vi "New (Single Trigger).vi"(6 "file name format (\"logfile_%<%Y-%m-%d_%H-%M-%S>T.log\")":string="logfile_%<%Y-%m-%d_%H-%M-%S>T.log", 7 "cleanup filter (never)":refnum<class "CleanupFilter.lvclass">, 8 "error in":errorcluster, 9 "rollover trigger (50 MB)":refnum<class "RolloverTrigger.lvclass">, 10 "formatter (JSON)":refnum<class "Formatter.lvclass">, 11 "log directory (<app dir>/logs)":path) -> (0 "error out":errorcluster, 2 "events":T1, 3 "file handler":refnum<class "File Handler.lvclass">)   [LabVIEW 2018, in "GLog.lvlib" / "File Handler.lvclass"]
doc: "Creates a new Handler which writes log records to a file."
uses:
  File Handler.lvclass
  C:/Users/Colin/Documents/software_projects/labview/glog/src/api/extension/formatting_handler_interface/Formatting Handler.lvclass
  extension/formatter_interface/Formatter.lvclass
  RolloverTrigger/RolloverTrigger.lvclass
  Events.ctl
  File Update Event.ctl
  CleanupFilter/CleanupFilter.lvclass
  File Handler.lvclass/File Handler.ctl
  extension/formatting_handler_interface/Formatting Handler.lvclass/Formatting Handler.ctl
  RolloverTrigger.Size/RolloverTrigger.Size.lvclass
  C:/Users/Colin/Documents/software_projects/labview/glog/src/api/configuration/handlers/file_handler/RolloverTrigger/RolloverTrigger.lvclass
  formatters/JSON_formatter/JSON.lvclass
  C:/Users/Colin/Documents/software_projects/labview/glog/src/api/extension/formatter_interface/Formatter.lvclass
  extension/formatting_handler_interface/Formatting Handler.lvclass
panel:
  # "Connector Pane"
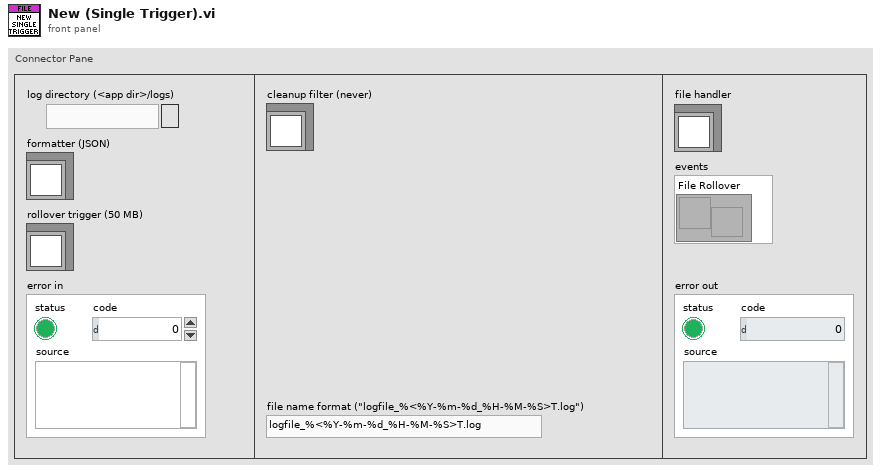
[diagram p1: front panel]
types:
  T1 = typedef "GLog.lvlib/File Handler.lvclass/Events.ctl" = cluster{"File Rollover":refnum<user-event>}
  T2 = typedef "GLog.lvlib/File Handler.lvclass/File Update Event.ctl" = cluster{"Current File":path, "Source":string}
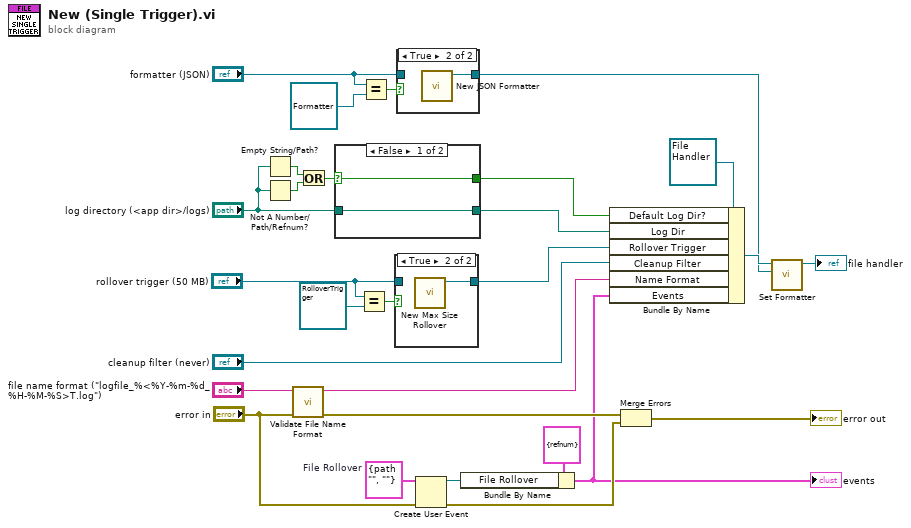
[diagram p0: block diagram]
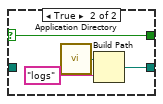
[diagram p4: hidden frame]
diagram:
  w16 = T2 {"Current File"=path "", "Source"=""}  # File Rollover
  n1 = Empty String/Path?(string/path="log directory (<app dir>/logs)") -> (empty?=w23:bool)
  n2 = Not A Number/Path/Refnum?(number/path/refnum="log directory (<app dir>/logs)") -> (NaN/Path/Refnum?=w27:bool)
  n3 = call "Validate File Name Format.vi"("error in"="error in", "name format in"="file name format (\"logfile_%<%Y-%m-%d_%H-%M-%S>T.log\")") -> ("error out"=w12:errorcluster, "name format out"=w8:string)  [unwired: 8 in]
  n4 = Or(x=w23, y=w27) -> (x .or. y?=w24:bool)
  n5 = case shown="False" w24 {
    selector: w24 -> [w29 w31]
    tunnel: "log directory (<app dir>/logs)" -> [w30 _]
    tunnel: [w30 w32] -> w26
    tunnel: [w29 w31] -> w1
    frame False {
    }
    frame True {
      n6 = call <vilib>:"Application Directory.vi"() -> ("Application Directory"=w34:path)
      n7 = Build Path(base path=w34, name or relative path="logs") -> (appended path=w32:path)
    }
  }
  n8 = Equal?(x="rollover trigger (50 MB)", y=refnum<class "RolloverTrigger.lvclass"> refnum ("GLog.lvlib:RolloverTrigger.lvclass")) -> (x = y?=w5:bool)
  n9 = Equal?(x="formatter (JSON)", y=refnum<class "Formatter.lvclass"> refnum ("formatter (JSON)")) -> (x = y?=w19:bool)
  n10 = case shown="True" w5 {
    tunnel: "rollover trigger (50 MB)" -> [w35 _]
    tunnel: [w35 w36] -> w2
    frame False {
    }
    frame True {
      n11 = call "New Max Size Rollover.vi"() -> ("size trigger"=w36:refnum<class "RolloverTrigger.Size.lvclass">)  [unwired: 11 in]
    }
  }
  n12 = case shown="True" w19 {
    tunnel: [w37 w38] -> w20
    tunnel: "formatter (JSON)" -> [w37 _]
    frame False {
    }
    frame True {
      n13 = call "New JSON Formatter.vi"() -> ("JSON formatter"=w38:refnum<class "JSON.lvclass">)  [unwired: 11 in]
    }
  }
  n14 = Create User Event(user event datatype=w16, error in="error in") -> (user event=w14:refnum<user-event>, error out=w10:errorcluster)
  n15 = Bundle By Name(cluster=T1 {"File Rollover"=refnum}, "File Rollover"=w14) -> (w7:T1)
  "events" <- w7
  n16 = Bundle By Name(cluster=refnum<class "File Handler.lvclass"> refnum ("file handler"), "Default Log Dir?"=w1, "Log Dir"=w26, "Rollover Trigger"=w2, "Cleanup Filter"="cleanup filter (never)", "Name Format"=w8, "Events"=w7) -> (w22:refnum<class "File Handler.lvclass">)
  n17 = Merge Errors(w12, w10) -> (→"error out":errorcluster)
  n18 = call "Set Formatter.vi"("formatter"=w20, "handler in"=w22) -> ("handler out"=→"file handler":refnum<class "File Handler.lvclass">)  [unwired: 9 in]
